vi "user32 SetWindowPos.vi"(0 "hWnd":u64, 1 "hWndInsertAfter":u64, 2 "X":i32, 3 "Y":i32, 4 "cx":i32, 5 "cy":i32, 6 "uFlags":u32=21, 7 "error in":errorcluster) -> (20 "return value":i32, 27 "error out":errorcluster)   [LabVIEW 2020, in "RemoteVI.lvlib"]
doc: "Moves and/or resizes the window hWnd and sets its Z order through user32.dll SetWindowPos (stdcall, called in any thread). X and Y are SCREEN pixels for a top-level window. uFlags 0x15 = SWP_NOSIZE | SWP_NOZORDER | SWP_NOACTIVATE moves the window only, without resizing, reordering or activating it - that is how RemoteVI Post Input.vi moves an open LabVIEW popup under the host cursor. return value is the Win32 BOOL: non-zero on success. When error in carries an error the DLL is not called. Generated by scripts\\Build Win32 Wrappers.vi - do not edit by hand, rebuild it."
uses:
  RemoteVI.lvlib
  user32.dll
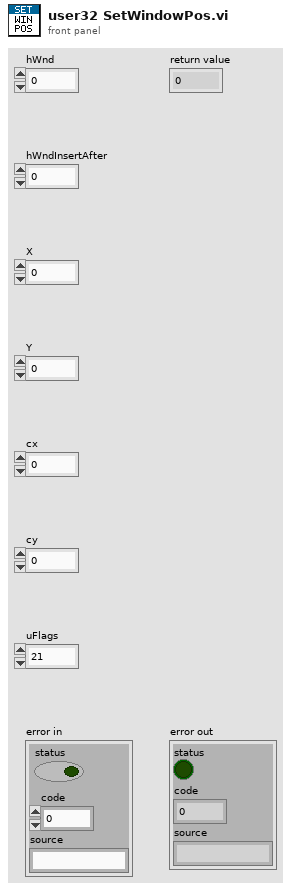
[diagram p1: front panel]
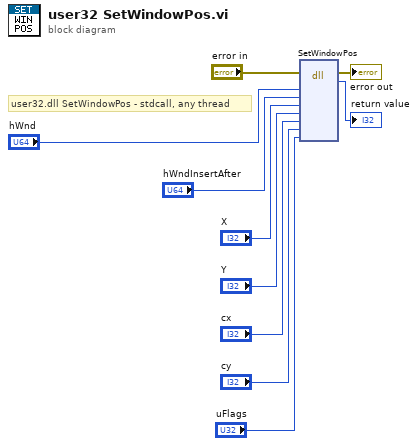
[diagram p0: block diagram]
diagram:
  # "user32.dll SetWindowPos - stdcall, any thread"
  n1 = dll-call lib="user32.dll" fn="SetWindowPos"(error in="error in", "hWnd"="hWnd", "hWndInsertAfter"="hWndInsertAfter", "X"="X", "Y"="Y", "cx"="cx", "cy"="cy", "uFlags"="uFlags") -> (error out=→"error out":errorcluster, →"return value":i32)  [unwired: 9 in, 1 out]
